vi "Test_status_bar.vi"(0 "Color Box  2":u32(colorbox), 3 "error out":errorcluster) -> (6 "Color Box":u32(colorbox), 9 "error out 2":errorcluster)   [LabVIEW 2021]
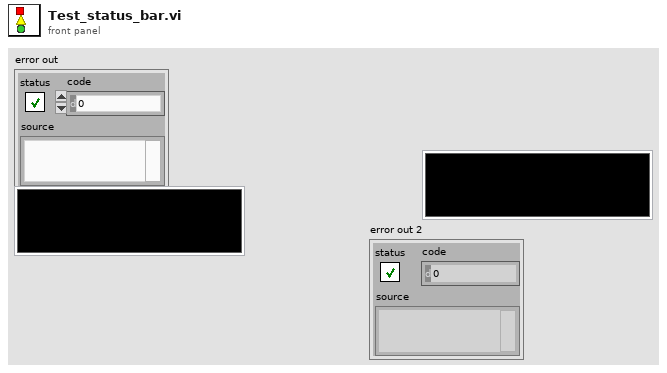
[diagram p1: front panel]
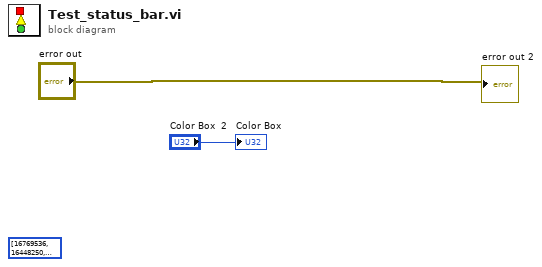
[diagram p0: block diagram]
diagram:
  (unwired) u32[] [16769536, 16448250, 16769536, 16777215, 16769536, 16777215, 16769536, 16579836, 16769536, 16711422, 16769536, 16777215, 16769536, 16777215, 16769536, 16382457, 16769536, 16645629, 16769536, 16711422, 16769536, 16579836, 16769536, 16579836, 16769536, 16777215, 16769536, 16777215, 16769536, 16777215, 16769536, 16777215, 16769536, 16777215, 16769536, 16645629, 16769536, 16777215, 16769536, 16777215]
  "error out 2" <- "error out"
  "Color Box" <- "Color Box  2"
